vi "140-2.vi"() -> ()   [LabVIEW 2025]
uses:
  <vilib>/Platform/TimedLoop/XDataNode/timing_clust.ctl
  <vilib>/Platform/TimedLoop/XDataNode/nitl_modes.ctl
  <vilib>/Platform/TimedLoop/XDataNode/wakeup.ctl
  <vilib>/eio/utilities/niEioResolveVilibRelativePath.vi
  <vilib>/rvi/interface/RandomDataEmulation/niFpgaRandomDataHandleErrors.vi
  <vilib>/rvi/Memory/Memory_Emulation/nirvimemoryFastEmulation.vi
  <vilib>/rvi/Memory/Memory_Emulation/nirvimemoryEmulation.vi
  <vilib>/rvi/Emulation/niFpgaEmulationIsFPGAContextNoSignature.vi
  <vilib>/rvi/DataTransferAndStorage/Container/Common/niFpgaContainerGetUniqueNameForEmu.vi
  <vilib>/rvi/Emulation/niFpgaProcessEmulError.vi
  <vilib>/rvi/Emulation/niFpgaSctlEmulationGetInTimedLoop.vi
  <vilib>/rvi/errors/nirviReportUnexpectedCaseInternalError (U32).vi
  <vilib>/rvi/Emulation/niFpgaEmulationReportErrorSimple.vi
  <vilib>/rvi/Emulation/niFpgaGetClockAttributes.vi
  <vilib>/rvi/Emulation/niFpgaCriticalErrorInLSC.vi
  <vilib>/rvi/linearAlgebra/MatrixMultiply/simVIs/SubVI/nifxpla_MatrixMultiply_SimMatrixSizes.vi
  <vilib>/rvi/linearAlgebra/MatrixMultiply/simVIs/SubVI/nifxpla_MatrixMultiply_Sim4WireAdapterVector.vi
  <vilib>/rvi/linearAlgebra/MatrixMultiply/simVIs/SubVI/nifxpla_MatrixMultiply_SimFrameHandShake.vi
  <vilib>/rvi/linearAlgebra/MatrixMultiply/simVIs/SubVI/nifxpla_MatrixMultiply_SimEndlessCounter.vi
  <vilib>/rvi/linearAlgebra/MatrixMultiply/simVIs/SubVI/nifxpla_MatrixMultiply_SimVectorDataBuffer.vi
  <vilib>/rvi/ClientSDK/Core/DevComputerLib/Private/Multiply(dfxp64).vi
  <vilib>/rvi/ClientSDK/Core/DevComputerLib/Private/Dfxp128ToDfxp256.vi
  <vilib>/rvi/ClientSDK/Core/DevComputerLib/Private/Add(dfxp256).vi
  <vilib>/rvi/ClientSDK/Core/DevComputerLib/Private/Subtract(dfxp256).vi
  <vilib>/rvi/ClientSDK/Core/DevComputerLib/Private/ToDfxp64(dfxp256).vi
  <vilib>/rvi/DataTransferAndStorage/Container/XNode/niFpgaContainer.xnode
  <vilib>/rvi/interface/RandomDataEmulation/nirviRandomDataFpgaReadWriteTemplate.vi
  <vilib>/platform/TimedLoop/XDataNode/XDataNode.xnode
  <vilib>/rvi/linearAlgebra/MatrixMultiply/XNode/nifxpla_MatrixMultiply.xnode
  <vilib>/rvi/linearAlgebra/MatrixMultiply/simVIs/nifxpla_MatrixMultiply_SimTemplateEinEout.vi
  <vilib>/rvi/linearAlgebra/MatrixMultiply/simVIs/nifxpla_MatrixMultiply_SimTemplateEinVout.vi
  <vilib>/rvi/linearAlgebra/MatrixMultiply/simVIs/nifxpla_MatrixMultiply_SimTemplateVinEout.vi
  <vilib>/rvi/linearAlgebra/MatrixMultiply/simVIs/nifxpla_MatrixMultiply_SimTemplateVinVout.vi
  <vilib>/Platform/TimedLoop/XDataNode/XDNodeRunTimeDep.lvlib
panel:
  out "Latency":u32
  out "Cycle Count":i32
  out "C1":fxp<+/-,32,16>[](array[numeric])
  out "C1+B":fxp<+/-,33,17>[](array[numeric])
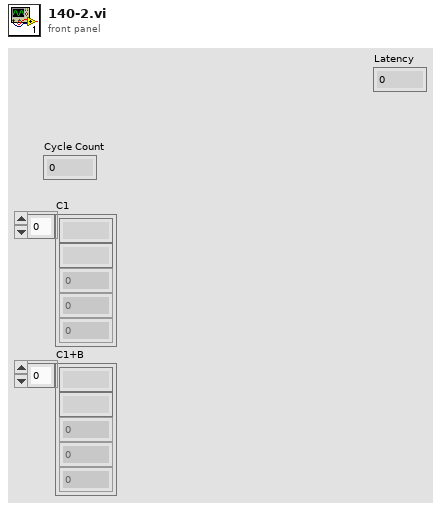
[diagram p1: front panel]
types:
  T1 = typedef "XDNodeRunTimeDep.lvlib/timing_clust.ctl" = cluster{"Expected End [f-1]":u64, "Actual End [f-1]":u64, "Finished Late? [f-1]":bool, "Expected End [i-1]":u64, "Actual End [i-1]":u64, "Finished Late? [i-1]":bool, "Expected Start [i]":u64, "Actual Start [i]":u64, "Expected Start [f]":u64, "Actual Start [f]":u64, "Source Name":string, "Structure Name":string, "Period":i64, "Deadline":i64, "Offset":i64, "Start":i64, "Priority":i32, "Timeout":i32, "Mode":T2, "Wakeup Reason":T3, "Error":errorcluster, "Source Type":string, "Secondary Source Type":string, "Global End Time":u64, "Global Start Time":u64, "Frame Duration":u64, "Iteration Duration":u64, "Assigned CPU":i32, "I/O Scan Engine Mode":u32}
  T2 = typedef "XDNodeRunTimeDep.lvlib/nitl_modes.ctl" = enum32{"No Change", "Process missed periods, maintain original phase", "Discard missed periods, maintain original phase", "Process missed periods, ignore original phase", "Discard missed periods, ignore original phase"}
  T3 = typedef "XDNodeRunTimeDep.lvlib/wakeup.ctl" = enum32{"Normal", "Aborted", "Asynchronous wakeup", "Timing source error", "Timed loop error", "Timeout"}
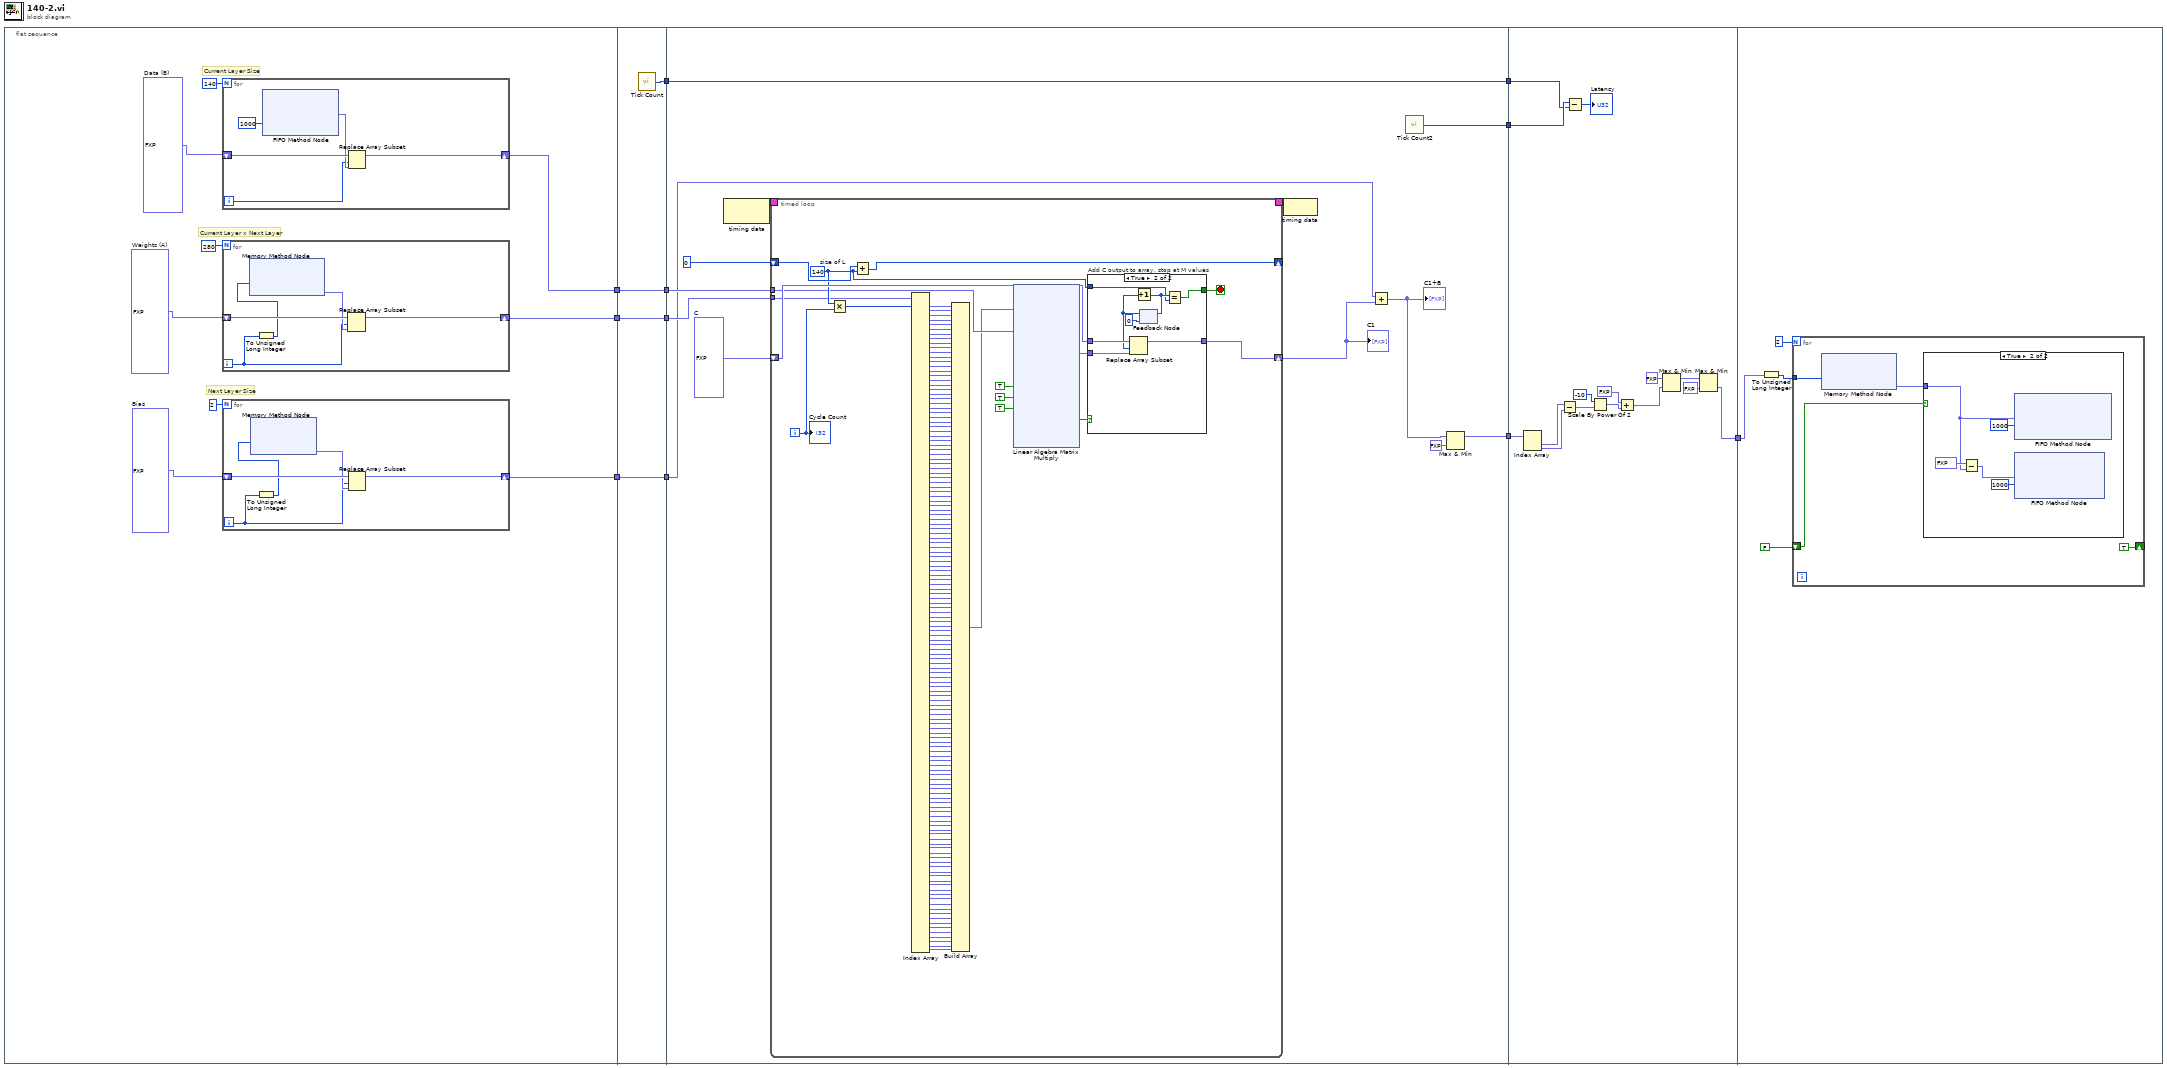
[diagram p0: block diagram]
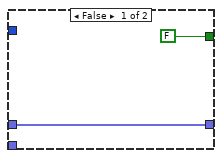
[diagram p2: hidden frame]
diagram:
  n1 = flat-sequence {
    tunnel: [w16] -> w7
    tunnel: [w13] -> w5
    tunnel: [w12] -> w2
    tunnel: [w39] -> w11
    tunnel: [w38] -> w8
    tunnel: w7 -> [w38]
    tunnel: [w37] -> w6
    tunnel: w5 -> [w37]
    tunnel: w2 -> [w36]
    tunnel: [w36] -> w1
    tunnel: [w52] -> w10
    tunnel: [w51] -> w9
    tunnel: [w49] -> w4
    tunnel: w11 -> [w52]
    tunnel: w8 -> [w43]
    tunnel: w6 -> [w40]
    tunnel: w1 -> [w41]
    tunnel: w10 -> [w236]
    tunnel: w9 -> [w237]
    tunnel: w4 -> [w234]
    tunnel: [w223] -> w3
    tunnel: w3 -> [w239]
    frame #0 {
      w14 = fxp<+/-,32,16>[] [0.0, 0.0]  # Bias
      w17 = fxp<+/-,32,16>[] [0.0, 0.0, 0.0, 0.0, 0.0, 0.0, 0.0, 0.0, 0.0, 0.0, 0.0, 0.0, 0.0, 0.0, 0.0, 0.0, 0.0, 0.0, 0.0, 0.0, 0.0, 0.0, 0.0, 0.0, 0.0, 0.0, 0.0, 0.0, 0.0, 0.0, 0.0, 0.0, 0.0, 0.0, 0.0, 0.0, 0.0, 0.0, 0.0, 0.0, 0.0, 0.0, 0.0, 0.0, 0.0, 0.0, 0.0, 0.0, 0.0, 0.0, 0.0, 0.0, 0.0, 0.0, 0.0, 0.0, 0.0, 0.0, 0.0, 0.0, 0.0, 0.0, 0.0, 0.0, 0.0, 0.0, 0.0, 0.0, 0.0, 0.0, 0.0, 0.0, 0.0, 0.0, 0.0, 0.0, 0.0, 0.0, 0.0, 0.0, 0.0, 0.0, 0.0, 0.0, 0.0, 0.0, 0.0, 0.0, 0.0, 0.0, 0.0, 0.0, 0.0, 0.0, 0.0, 0.0, 0.0, 0.0, 0.0, 0.0, 0.0, 0.0, 0.0, 0.0, 0.0, 0.0, 0.0, 0.0, 0.0, 0.0, 0.0, 0.0, 0.0, 0.0, 0.0, 0.0, 0.0, 0.0, 0.0, 0.0, 0.0, 0.0, 0.0, 0.0, 0.0, 0.0, 0.0, 0.0, 0.0, 0.0, 0.0, 0.0, 0.0, 0.0, 0.0, 0.0, 0.0, 0.0, 0.0, 0.0, 0.0, 0.0, 0.0, 0.0, 0.0, 0.0, 0.0, 0.0, 0.0, 0.0, 0.0, 0.0, 0.0, 0.0, 0.0, 0.0, 0.0, 0.0, 0.0, 0.0, 0.0, 0.0, 0.0, 0.0, 0.0, 0.0, 0.0, 0.0, 0.0, 0.0, 0.0, 0.0, 0.0, 0.0, 0.0, 0.0, 0.0, 0.0, 0.0, 0.0, 0.0, 0.0, 0.0, 0.0, 0.0, 0.0, 0.0, 0.0, 0.0, 0.0, 0.0, 0.0, 0.0, 0.0, 0.0, 0.0, 0.0, 0.0, 0.0, 0.0, 0.0, 0.0, 0.0, 0.0, 0.0, 0.0, 0.0, 0.0, 0.0, 0.0, 0.0, 0.0, 0.0, 0.0, 0.0, 0.0, 0.0, 0.0, 0.0, 0.0, 0.0, 0.0, 0.0, 0.0, 0.0, 0.0, 0.0, 0.0, 0.0, 0.0, 0.0, 0.0, 0.0, 0.0, 0.0, 0.0, 0.0, 0.0, 0.0, 0.0, 0.0, 0.0, 0.0, 0.0, 0.0, 0.0, 0.0, 0.0, 0.0, 0.0, 0.0, 0.0, 0.0, 0.0, 0.0, 0.0, 0.0, 0.0, 0.0, 0.0, 0.0, 0.0, 0.0, 0.0, 0.0, 0.0, 0.0, 0.0, 0.0, 0.0, 0.0, 0.0, 0.0, 0.0, 0.0, 0.0, 0.0, 0.0, 0.0, 0.0]  # Weights (A)
      w19 = fxp<+/-,32,16>[] [0.0, 0.0, 0.0, 0.0, 0.0, 0.0, 0.0, 0.0, 0.0, 0.0, 0.0, 0.0, 0.0, 0.0, 0.0, 0.0, 0.0, 0.0, 0.0, 0.0, 0.0, 0.0, 0.0, 0.0, 0.0, 0.0, 0.0, 0.0, 0.0, 0.0, 0.0, 0.0, 0.0, 0.0, 0.0, 0.0, 0.0, 0.0, 0.0, 0.0, 0.0, 0.0, 0.0, 0.0, 0.0, 0.0, 0.0, 0.0, 0.0, 0.0, 0.0, 0.0, 0.0, 0.0, 0.0, 0.0, 0.0, 0.0, 0.0, 0.0, 0.0, 0.0, 0.0, 0.0, 0.0, 0.0, 0.0, 0.0, 0.0, 0.0, 0.0, 0.0, 0.0, 0.0, 0.0, 0.0, 0.0, 0.0, 0.0, 0.0, 0.0, 0.0, 0.0, 0.0, 0.0, 0.0, 0.0, 0.0, 0.0, 0.0, 0.0, 0.0, 0.0, 0.0, 0.0, 0.0, 0.0, 0.0, 0.0, 0.0, 0.0, 0.0, 0.0, 0.0, 0.0, 0.0, 0.0, 0.0, 0.0, 0.0, 0.0, 0.0, 0.0, 0.0, 0.0, 0.0, 0.0, 0.0, 0.0, 0.0, 0.0, 0.0, 0.0, 0.0, 0.0, 0.0, 0.0, 0.0, 0.0, 0.0, 0.0, 0.0, 0.0, 0.0, 0.0, 0.0, 0.0, 0.0, 0.0, 0.0]  # Data (B)
      # "Next Layer Size"
      # "Current Layer Size"
      # "Current Layer x Next Layer"
      n2 = for {
        N: 280 -> [_]
        shift-right: [w29] -> w12
        shift-left: w17 -> [w30]
        i -> [w27]
        n3 = To Unsigned Long Integer(number=w27) -> (unsigned 32bit integer=w26:u32)
        n4 = xnode ("Memory Method Node")("Address"=w26) -> ("Data"=w28:fxp<+/-,32,16>)  [unwired: 1 in, 1 out]
        n5 = Replace Array Subset(array=w30, new element=w28, index=w27) -> (w29:fxp<+/-,32,16>[])
      }
      n6 = for {
        N: 140 -> [_]
        shift-right: [w32] -> w16
        shift-left: w19 -> [w34]
        i -> [w31]
        n7 = xnode ("FIFO Method Node")("Timeout"=1000) -> ("Element"=w33:fxp<+/-,32,16>)  [unwired: 1 in, 2 out]
        n8 = Replace Array Subset(array=w34, new element=w33, index=w31) -> (w32:fxp<+/-,32,16>[])
      }
      n9 = for {
        N: 2 -> [_]
        shift-right: [w24] -> w13
        shift-left: w14 -> [w25]
        i -> [w22]
        n10 = To Unsigned Long Integer(number=w22) -> (unsigned 32bit integer=w21:u32)
        n11 = xnode ("Memory Method Node")("Address"=w21) -> ("Data"=w23:fxp<+/-,32,16>)  [unwired: 1 in, 1 out]
        n12 = Replace Array Subset(array=w25, new element=w23, index=w22) -> (w24:fxp<+/-,32,16>[])
      }
    }
    frame #1 {
      n13 = call "Tick Count"() -> ("Tick Count(Ticks)"=w39:u32)
    }
    frame #2 {
      w46 = fxp<+/-,32,16>[] [0.0, 0.0]  # C
      n14 = node-c288() -> (w48:T1)  [unwired: 1 in]
      n15 = timed-loop {
        timing: w48 -> [_]
        timing-out: [_] -> w47
        shift-right: [w207] -> w44
        shift-left: w46 -> [w206]
        shift-right: [w200] -> _
        shift-left: 0 ("length") -> [w201]
        tunnel: w41 -> [w67]
        tunnel: w43 -> [w66]
        i -> [w187]
        stop <- w205 stop-if-true
        w186 = 140  # size of L
        n16 = Multiply(x=w186, y=w187) -> (x*y=w198:i32)
        n17 = Add(x=w201, y=w186) -> (x+y=w200:i32)
        n18 = Index Array(array=w67, index #1=w198) -> (element #1=w197:fxp<+/-,32,16>, element #2=w196:fxp<+/-,32,16>, element #3=w195:fxp<+/-,32,16>, element #4=w194:fxp<+/-,32,16>, element #5=w193:fxp<+/-,32,16>, element #6=w192:fxp<+/-,32,16>, element #7=w191:fxp<+/-,32,16>, element #8=w190:fxp<+/-,32,16>, element #9=w189:fxp<+/-,32,16>, element #10=w188:fxp<+/-,32,16>, element #11=w185:fxp<+/-,32,16>, element #12=w184:fxp<+/-,32,16>, element #13=w183:fxp<+/-,32,16>, element #14=w182:fxp<+/-,32,16>, element #15=w181:fxp<+/-,32,16>, element #16=w180:fxp<+/-,32,16>, element #17=w179:fxp<+/-,32,16>, element #18=w178:fxp<+/-,32,16>, element #19=w177:fxp<+/-,32,16>, element #20=w176:fxp<+/-,32,16>, element #21=w175:fxp<+/-,32,16>, element #22=w174:fxp<+/-,32,16>, element #23=w173:fxp<+/-,32,16>, element #24=w172:fxp<+/-,32,16>, element #25=w171:fxp<+/-,32,16>, element #26=w170:fxp<+/-,32,16>, element #27=w169:fxp<+/-,32,16>, element #28=w168:fxp<+/-,32,16>, element #29=w167:fxp<+/-,32,16>, element #30=w166:fxp<+/-,32,16>, element #31=w165:fxp<+/-,32,16>, element #32=w164:fxp<+/-,32,16>, element #33=w163:fxp<+/-,32,16>, element #34=w161:fxp<+/-,32,16>, element #35=w162:fxp<+/-,32,16>, element #36=w160:fxp<+/-,32,16>, element #37=w159:fxp<+/-,32,16>, element #38=w158:fxp<+/-,32,16>, element #39=w157:fxp<+/-,32,16>, element #40=w156:fxp<+/-,32,16>, element #41=w155:fxp<+/-,32,16>, element #42=w154:fxp<+/-,32,16>, element #43=w153:fxp<+/-,32,16>, element #44=w152:fxp<+/-,32,16>, element #45=w150:fxp<+/-,32,16>, element #46=w151:fxp<+/-,32,16>, element #47=w149:fxp<+/-,32,16>, element #48=w148:fxp<+/-,32,16>, element #49=w147:fxp<+/-,32,16>, element #50=w146:fxp<+/-,32,16>, element #51=w145:fxp<+/-,32,16>, element #52=w144:fxp<+/-,32,16>, element #53=w143:fxp<+/-,32,16>, element #54=w142:fxp<+/-,32,16>, element #55=w141:fxp<+/-,32,16>, element #56=w140:fxp<+/-,32,16>, element #57=w138:fxp<+/-,32,16>, element #58=w139:fxp<+/-,32,16>, element #59=w137:fxp<+/-,32,16>, element #60=w136:fxp<+/-,32,16>, element #61=w135:fxp<+/-,32,16>, element #62=w134:fxp<+/-,32,16>, element #63=w133:fxp<+/-,32,16>, element #64=w132:fxp<+/-,32,16>, element #65=w131:fxp<+/-,32,16>, element #66=w129:fxp<+/-,32,16>, element #67=w130:fxp<+/-,32,16>, element #68=w127:fxp<+/-,32,16>, element #69=w128:fxp<+/-,32,16>, element #70=w125:fxp<+/-,32,16>, element #71=w126:fxp<+/-,32,16>, element #72=w123:fxp<+/-,32,16>, element #73=w124:fxp<+/-,32,16>, element #74=w122:fxp<+/-,32,16>, element #75=w121:fxp<+/-,32,16>, element #76=w120:fxp<+/-,32,16>, element #77=w119:fxp<+/-,32,16>, element #78=w118:fxp<+/-,32,16>, element #79=w117:fxp<+/-,32,16>, element #80=w116:fxp<+/-,32,16>, element #81=w115:fxp<+/-,32,16>, element #82=w114:fxp<+/-,32,16>, element #83=w113:fxp<+/-,32,16>, element #84=w112:fxp<+/-,32,16>, element #85=w110:fxp<+/-,32,16>, element #86=w111:fxp<+/-,32,16>, element #87=w109:fxp<+/-,32,16>, element #88=w107:fxp<+/-,32,16>, element #89=w108:fxp<+/-,32,16>, element #90=w106:fxp<+/-,32,16>, element #91=w105:fxp<+/-,32,16>, element #92=w104:fxp<+/-,32,16>, element #93=w103:fxp<+/-,32,16>, element #94=w102:fxp<+/-,32,16>, element #95=w101:fxp<+/-,32,16>, element #96=w100:fxp<+/-,32,16>, element #97=w99:fxp<+/-,32,16>, element #98=w98:fxp<+/-,32,16>, element #99=w97:fxp<+/-,32,16>, element #100=w96:fxp<+/-,32,16>, element #101=w95:fxp<+/-,32,16>, element #102=w94:fxp<+/-,32,16>, element #103=w93:fxp<+/-,32,16>, element #104=w92:fxp<+/-,32,16>, element #105=w91:fxp<+/-,32,16>, element #106=w90:fxp<+/-,32,16>, element #107=w89:fxp<+/-,32,16>, element #108=w88:fxp<+/-,32,16>, element #109=w87:fxp<+/-,32,16>, element #110=w85:fxp<+/-,32,16>, element #111=w86:fxp<+/-,32,16>, element #112=w83:fxp<+/-,32,16>, element #113=w84:fxp<+/-,32,16>, element #114=w82:fxp<+/-,32,16>, element #115=w80:fxp<+/-,32,16>, element #116=w81:fxp<+/-,32,16>, element #117=w79:fxp<+/-,32,16>, element #118=w78:fxp<+/-,32,16>, element #119=w77:fxp<+/-,32,16>, element #120=w76:fxp<+/-,32,16>, element #121=w75:fxp<+/-,32,16>, element #122=w74:fxp<+/-,32,16>, element #123=w73:fxp<+/-,32,16>, element #124=w72:fxp<+/-,32,16>, element #125=w71:fxp<+/-,32,16>, element #126=w70:fxp<+/-,32,16>, element #127=w69:fxp<+/-,32,16>, element #128=w68:fxp<+/-,32,16>, element #129=w63:fxp<+/-,32,16>, element #130=w64:fxp<+/-,32,16>, element #131=w62:fxp<+/-,32,16>, element #132=w61:fxp<+/-,32,16>, element #133=w60:fxp<+/-,32,16>, element #134=w59:fxp<+/-,32,16>, element #135=w58:fxp<+/-,32,16>, element #136=w57:fxp<+/-,32,16>, element #137=w56:fxp<+/-,32,16>, element #138=w55:fxp<+/-,32,16>, element #139=w54:fxp<+/-,32,16>, element #140=w53:fxp<+/-,32,16>)  [unwired: 139 in]
        n19 = Build Array(w197, w196, w195, w194, w193, w192, w191, w190, w189, w188, w185, w184, w183, w182, w181, w180, w179, w178, w177, w176, w175, w174, w173, w172, w171, w170, w169, w168, w167, w166, w165, w164, w163, w161, w162, w160, w159, w158, w157, w156, w155, w154, w153, w152, w150, w151, w149, w148, w147, w146, w145, w144, w143, w142, w141, w140, w138, w139, w137, w136, w135, w134, w133, w132, w131, w129, w130, w127, w128, w125, w126, w123, w124, w122, w121, w120, w119, w118, w117, w116, w115, w114, w113, w112, w110, w111, w109, w107, w108, w106, w105, w104, w103, w102, w101, w100, w99, w98, w97, w96, w95, w94, w93, w92, w91, w90, w89, w88, w87, w85, w86, w83, w84, w82, w80, w81, w79, w78, w77, w76, w75, w74, w73, w72, w71, w70, w69, w68, w63, w64, w62, w61, w60, w59, w58, w57, w56, w55, w54, w53) -> (w65:fxp<+/-,32,16>[])
        n20 = xnode ("Linear Algebra Matrix Multiply")("ar"=w65, "br"=w66, "a valid"=TRUE, "b valid"=TRUE, "ready for output (T)"=TRUE) -> ("cr"=w203:fxp<+/-,64,40>[], "output valid"=w199:bool)  [unwired: 2 in, 4 out]
        n21 = case "Add C output to array, stop at M values" shown="True" w199 {
          tunnel: w203 -> [_ w214]
          tunnel: [w210 w217] -> w207
          tunnel: w206 -> [w210 w218]
          tunnel: [FALSE w215] -> w205
          tunnel: w186 -> [_ w211]
          frame False {
          }
          frame True {
            n22 = feedback #1(0 ("x")) -> (w213:i32)
            n23 = Replace Array Subset(array=w218, new element=w214, index=w213) -> (w217:fxp<+/-,32,16>[])
            n24 = Increment(x=w213) -> (x+1=w212:i32)
            n25 = feedback-in #1(w212) -> ()
            n26 = Equal?(x=w212, y=w211) -> (x = y?=w215:bool)
          }
        }
        "Cycle Count" <- w187
      }
      "C1" <- w44
      n27 = node-c288(w47) -> ()
      n28 = Add(x=w40, y=w44) -> (x+y=w42:fxp<+/-,33,17>[])
      "C1+B" <- w42
      n29 = call "Tick Count2"() -> ("Tick Count(Ticks)"=w51:u32)
      n30 = Max & Min(x=w42, y=fxp<+,1,1> 0.0) -> (max(x,y)=w49:fxp<+/-,33,17>[])  [unwired: 1 out]
    }
    frame #3 {
      n31 = Index Array(array=w234) -> (element #1=w225:fxp<+/-,33,17>, element #2=w224:fxp<+/-,33,17>)  [unwired: 2 in]
      n32 = Subtract(x=w225, y=w224) -> (x-y=w230:fxp<+/-,34,18>)
      n33 = Subtract(x=w237, y=w236) -> (x-y=→"Latency":u32)
      n34 = Scale By Power Of 2(n=i16 -10, x=w230) -> (x*2^n=w231:fxp<+/-,34,18>)
      n35 = Add(x=fxp<+,1,9> 256.0, y=w231) -> (x+y=w232:fxp<+/-,35,19>)
      n36 = Max & Min(x=fxp<+,1,1> 0.0, y=w232) -> (max(x,y)=w233:fxp<+/-,35,19>)  [unwired: 1 out]
      n37 = Max & Min(x=w233, y=fxp<+,9,9> 511.0) -> (min(x,y)=w223:fxp<+/-,35,19>)  [unwired: 1 out]
    }
    frame #4 {
      n38 = To Unsigned Long Integer(number=w239) -> (unsigned 32bit integer=w238:u32)
      n39 = for {
        N: 2 -> [_]
        tunnel: w238 -> [w245]
        shift-right: [TRUE] -> _
        shift-left: FALSE -> [w244]
        n40 = xnode ("Memory Method Node")("Address"=w245) -> ("Data"=w242:fxp<+/-,32,16>)  [unwired: 1 in, 1 out]
        n41 = case shown="True" w244 {
          tunnel: w242 -> [_ w246]
          frame False {
          }
          frame True {
            n42 = Subtract(x=fxp<+,1,16> 32768.0, y=w246) -> (x-y=w250:fxp<+,33,17>)
            n43 = xnode ("FIFO Method Node")("Element"=w246, "Timeout"=1000) -> ()  [unwired: 1 in, 2 out]
            n44 = xnode ("FIFO Method Node")("Element"=w250, "Timeout"=1000) -> ()  [unwired: 1 in, 2 out]
          }
        }
      }
    }
  }
